vi "Get Item Count.vi"(8 "error in (no error)":errorcluster) -> (0 "error out":errorcluster, 3 "OUT":u32)   [LabVIEW 2017, in "HID_ARZ.lvlib"]
doc: "GET_ITEM_COUNT GetItemCount;"
uses:
  HID_ARZ.lvlib
  <userlib>/HID_ARZ/mcHID.dll
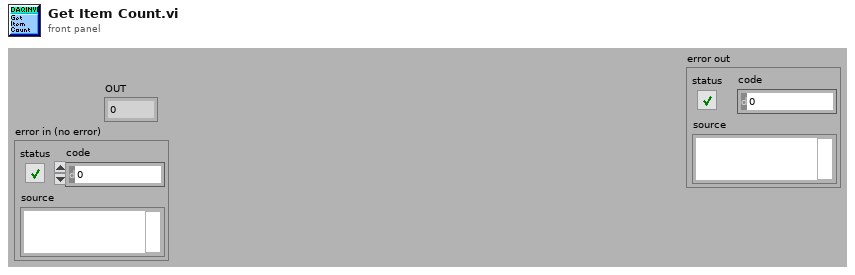
[diagram p1: front panel]
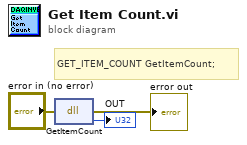
[diagram p0: block diagram]
diagram:
  # "GET_ITEM_COUNT GetItemCount;"
  n1 = dll-call lib="C:/Program Files (x86)/National Instruments/LabVIEW 2017/user.lib/HID_ARZ/mcHID.*" fn="GetItemCount"(error in="error in (no error)") -> (error out=→"error out":errorcluster, "return type"=→"OUT":u32)  [unwired: 2 in, 1 out]
